vi "Launch Executor.vi"(5 "Results Folder":path, 7 "Stopped Notification":refnum<notifier>, 8 "error in":errorcluster, 11 "Displays":T1) -> (0 "error out":errorcluster, 3 "Enqueuer":refnum<class "Message Enqueuer.lvclass">)   [LabVIEW 2026, in "Sequence Executor.lvclass"]
doc: "Static. Configures the executor (off-pane Executor seed, display refs bundle, notifier, results folder) and launches it as root; returns its Message Enqueuer."
uses:
  Sequence Executor.lvclass
  <vilib>/ActorFramework/Message Enqueuer/Message Enqueuer.lvclass
  <vilib>/ActorFramework/Actor/Actor.lvclass
panel:
  in  "Executor seed":refnum<class "Sequence Executor.lvclass">
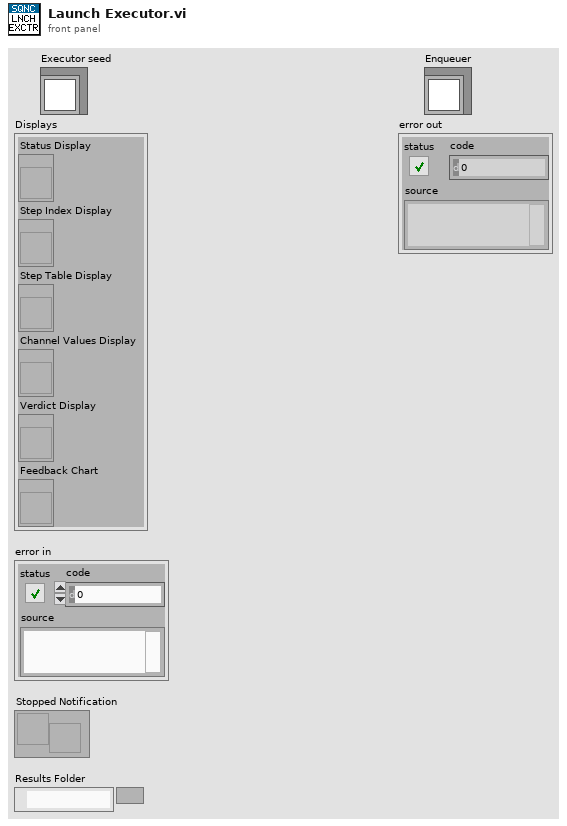
[diagram p1: front panel]
types:
  T1 = cluster{"Status Display":refnum<vi>, "Step Index Display":refnum<vi>, "Step Table Display":refnum<vi>, "Channel Values Display":refnum<vi>, "Verdict Display":refnum<vi>, "Feedback Chart":refnum<vi>}
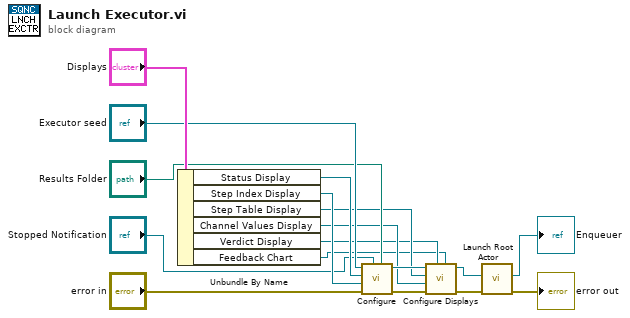
[diagram p0: block diagram]
diagram:
  n1 = Unbundle By Name("Displays") -> ("Status Display"=w15:refnum<vi>, "Step Index Display"=w14:refnum<vi>, "Step Table Display"=w9:refnum<vi>, "Channel Values Display"=w8:refnum<vi>, "Verdict Display"=w6:refnum<vi>, "Feedback Chart"=w5:refnum<vi>)
  n2 = call "Configure.vi"("Results Folder"="Results Folder", "Stopped Notification"="Stopped Notification", "error in"="error in", "Step Index Display"=w14, "Status Display"=w15, "Sequence Executor in"="Executor seed") -> ("error out"=w7:errorcluster, "Sequence Executor out"=w10:refnum<class "Sequence Executor.lvclass">)  [unwired: 4 in]
  n3 = call "Configure Displays.vi"("Feedback Chart"=w5, "Verdict Display"=w6, "error in"=w7, "Channel Values Display"=w8, "Step Table Display"=w9, "Sequence Executor in"=w10) -> ("error out"=w3:errorcluster, "Sequence Executor out"=w4:refnum<class "Sequence Executor.lvclass">)  [unwired: 4 in]
  n4 = call <vilib>:"Launch Root Actor.vi"("error in (no error)"=w3, "Actor"=w4) -> ("error out"=→"error out":errorcluster, "Actor's Enqueuer"=→"Enqueuer":refnum<class "Message Enqueuer.lvclass">)  [unwired: 8 in]
